vi "Actor Core.vi"(8 "error in":errorcluster, 11 "Basic SPIM Controller in":refnum<class "Basic SPIM Controller.lvclass">) -> (0 "error out":errorcluster, 3 "Actor out":refnum<class "Actor.lvclass">)   [LabVIEW 2020, in "DAQ Timed SPIM.lvlib" / "Basic SPIM Controller.lvclass"]
doc: "(<B>Filename</B>: Actor Framework.lvlib:Actor.lvclass:Actor Core.vi)\n\nReceives messages to the actor, reacts to them, and initiates any error handling that may shut the actor down.\n\nDescendant classes may override this VI to append parallel tasks for the actor to complete while it handles messages. Overrides use the Call Parent Class Method node."
uses:
  Basic SPIM Controller.lvclass
  C:/Program Files/National Instruments/LabVIEW 2020/vi.lib/ActorFramework/Actor/Actor.lvclass
  <vilib>/ActorFramework/Actor/Actor.lvclass
  <vilib>/ActorFramework/Actor/Actor.lvclass/Actor.ctl
  <vilib>/ActorFramework/Message Enqueuer/Message Enqueuer.lvclass/Message Enqueuer.ctl
  DAQ Timed SPIM Messages/Start Triggered Acq Msg/Start Triggered Acq Msg.lvclass/Start Triggered Acq Msg.ctl
  <vilib>/ActorFramework/Message Enqueuer/Init from Existing Queue.vi
  <vilib>/ActorFramework/Message Enqueuer/Enqueue.vi
  DAQ Timed SPIM Messages/Stop Triggered Acq Msg/Stop Triggered Acq Msg.lvclass
  C:/Program Files/National Instruments/LabVIEW 2020/vi.lib/ActorFramework/Message/Message.lvclass
  DAQ Timed SPIM Messages/Start Triggered Acq Msg/Start Triggered Acq Msg.lvclass
  <vilib>/ActorFramework/Stop Msg/Stop Msg.lvclass
  <vilib>/ActorFramework/Message Priority Queue/Priority Enqueue.vi
  <vilib>/ActorFramework/Message Enqueuer/Message Enqueuer.lvclass
panel:
  in  "Stop Button":bool
  in  "Stop Signal":bool
  in  "Run Button":bool
  in  "Record Button":bool
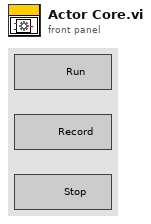
[diagram p1: front panel]
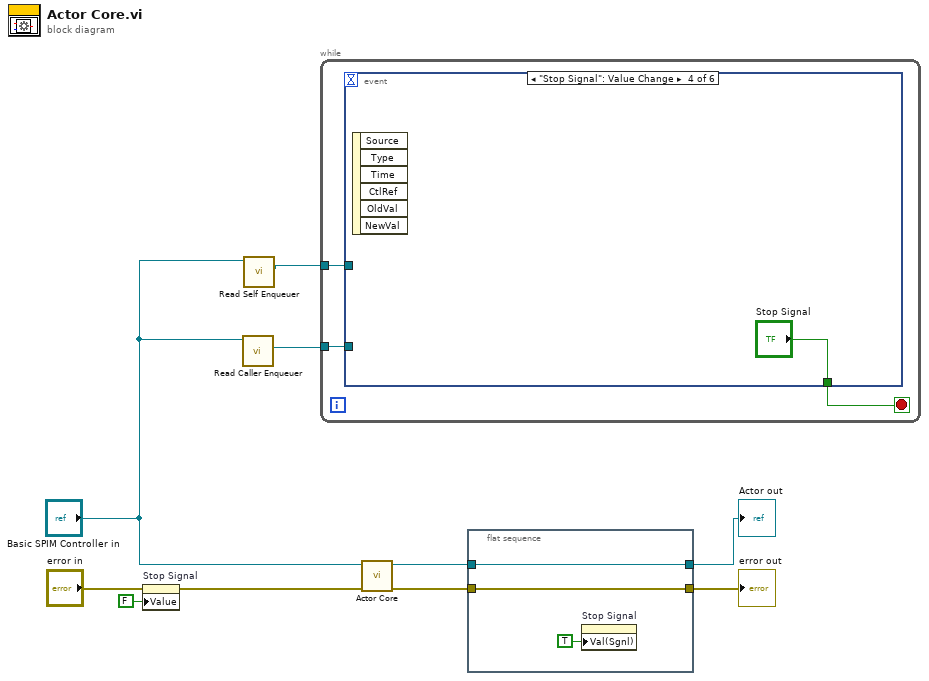
[diagram p0: block diagram]
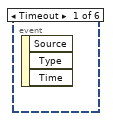
[diagram p2: hidden frame]
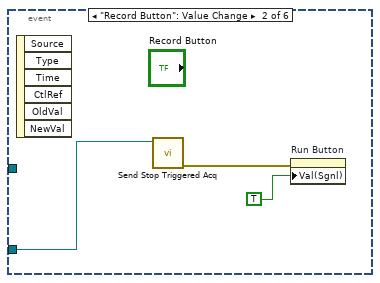
[diagram p3: hidden frame]
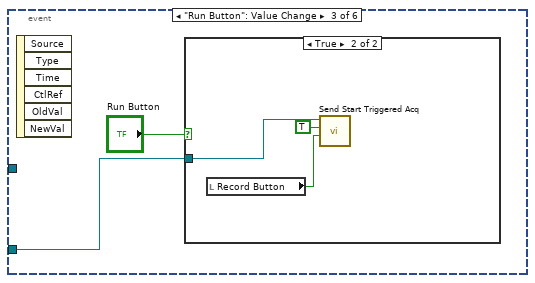
[diagram p4: hidden frame]
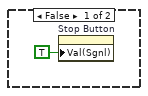
[diagram p5: hidden frame]
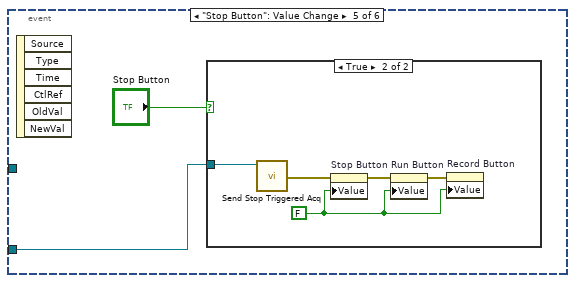
[diagram p6: hidden frame]
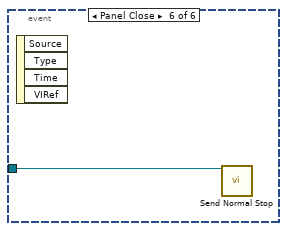
[diagram p8: hidden frame]
diagram:
  n1 = property on="Stop Signal" class="Bool (strict)"(error in="error in", "Value"=FALSE ("Stop Signal")) -> (error out=w6:errorcluster)  [unwired: 1 in, 1 out]
  n2 = call <vilib>:"Read Caller Enqueuer.vi"("Actor"="Basic SPIM Controller in") -> ("Caller Enqueuer"=w10:refnum<class "Message Enqueuer.lvclass">)  [unwired: 10 in]
  n3 = call <vilib>:"Read Self Enqueuer.vi"("Actor"="Basic SPIM Controller in") -> ("Self Enqueuer"=w9:refnum<class "Message Enqueuer.lvclass">)  [unwired: 10 in]
  n4 = while {
    tunnel: w10 -> [w13]
    tunnel: w9 -> [w11]
    stop <- w12 stop-if-true
    n5 = event shown="[3] \"Stop Signal\": Value Change" {
      selector: _ -> [_ _ _ _ _ _]
      dyn-events: _ -> [_ _ _ _ _ _]
      timeout: _ -> [_ _ _ _ _ _]
      tunnel: w13 -> [_ w16 w17 _ w25 _]
      tunnel: [_ _ _ "Stop Signal" _ _] -> w12
      tunnel: w11 -> [_ _ _ _ _ w31]
      event Timeout {
        n6 = event-data() -> ()  [unwired: 1 in, 3 out]
      }
      event "Record Button": Value Change {
        n7 = event-data() -> ()  [unwired: 1 in, 6 out]
        n8 = call "Send Stop Triggered Acq.vi"("Message Enqueuer"=w16) -> ("error out"=w15:errorcluster)  [unwired: 9 in, 1 out]
        n9 = property on="Run Button" class="Bool (strict)"(error in=w15, "Val(Sgnl)"=TRUE ("Value (Signaling)")) -> ()  [unwired: 1 in, 2 out]
      }
      event "Run Button": Value Change {
        n10 = event-data() -> ()  [unwired: 1 in, 6 out]
        n11 = case shown="True" "Run Button" {
          tunnel: w17 -> [_ w22]
          frame False {
            n12 = property on="Stop Button" class="Bool (strict)"("Val(Sgnl)"=TRUE ("Value (Signaling)")) -> ()  [unwired: 2 in, 2 out]
          }
          frame True {
            n13 = local read "Record Button"() -> (w20:bool)
            n14 = call "Send Start Triggered Acq.vi"("Write to disk?"=w20, "Repeat?"=TRUE, "Message Enqueuer"=w22) -> ()  [unwired: 7 in, 2 out]
          }
        }
      }
      event "Stop Signal": Value Change {
        n15 = event-data() -> ()  [unwired: 1 in, 6 out]
      }
      event "Stop Button": Value Change {
        n16 = event-data() -> ()  [unwired: 1 in, 6 out]
        n17 = case shown="True" "Stop Button" {
          tunnel: w25 -> [_ w30]
          frame False {
          }
          frame True {
            w28 = FALSE ("Stop Button")
            n18 = call "Send Stop Triggered Acq.vi"("Message Enqueuer"=w30) -> ("error out"=w29:errorcluster)  [unwired: 9 in, 1 out]
            n19 = property on="Stop Button" class="Bool (strict)"(error in=w29, "Value"=w28) -> (error out=w27:errorcluster)  [unwired: 1 in, 1 out]
            n20 = property on="Run Button" class="Bool (strict)"(error in=w27, "Value"=w28) -> (error out=w26:errorcluster)  [unwired: 1 in, 1 out]
            n21 = property on="Record Button" class="Bool (strict)"(error in=w26, "Value"=w28) -> ()  [unwired: 1 in, 2 out]
          }
        }
      }
      event Panel Close {
        n22 = event-data() -> ()  [unwired: 1 in, 4 out]
        n23 = call <vilib>:"Send Normal Stop.vi"("Message Enqueuer"=w31) -> ()  [unwired: 10 in, 1 out]
      }
    }
  }
  n24 = call-parent "Actor Core.vi"("error in"=w6, "Actor in"="Basic SPIM Controller in") -> ("error out"=w2:errorcluster, "Actor out"=w4:refnum<class "Actor.lvclass">)  [unwired: 8 in]
  n25 = flat-sequence {
    tunnel: w4 -> [w34]
    tunnel: [w34] -> w3
    tunnel: w2 -> [w33]
    tunnel: [w33] -> w1
    frame #0 {
      n26 = property on="Stop Signal" class="Bool (strict)"("Val(Sgnl)"=TRUE ("Value (Signaling)")) -> ()  [unwired: 2 in, 2 out]
    }
  }
  "error out" <- w1
  "Actor out" <- w3
